vi "Initialization.vi"(8 "error in":errorcluster, 9 "UI Refs":T1, 10 "user event":T2, 11 "F18 Blowdown":refnum<class "F18 Blowdown.lvclass">) -> (0 "error out":errorcluster, 3 "F18 Blowdown OUT":refnum<class "F18 Blowdown.lvclass">)   [LabVIEW 2025, in "F18 Blowdown.lvlib" / "F18 Blowdown.lvclass"]
uses:
  F18 Blowdown.lvclass
  Users/Public/Documents/Sandia National Labs/TSS Plugin/CEF.lvlibp/Node/UserEventRef.ctl
  Users/Public/Documents/Sandia National Labs/TSS Plugin/Tests/XY Plotter.lvlibp/XY  Plotter/XY Plotter.lvclass
  F18 Blowdown.lvclass/F18 Blowdown.ctl
  Users/Public/Documents/Sandia National Labs/TSS Plugin/CEF.lvlibp/Node/CEF_Node.lvclass
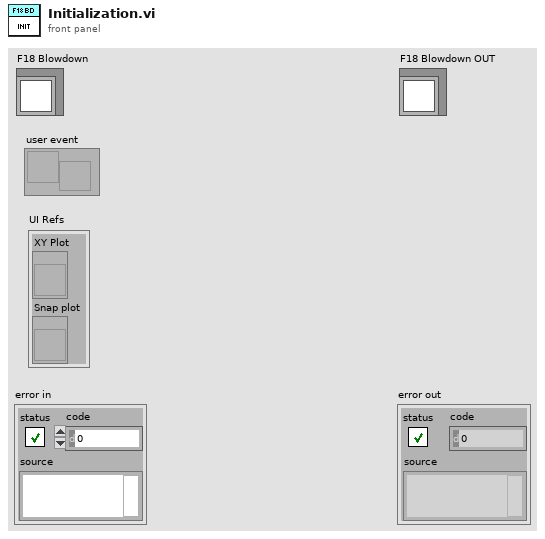
[diagram p1: front panel]
types:
  T1 = cluster{"XY Plot":refnum<vi>, "Snap plot":refnum<vi>}
  T2 = typedef "CEF.lvlibp/CEF_Node.lvclass/UserEventRef.ctl" = refnum<user-event>
  T3 = cluster{"Name":string, "Color":u32, "Style":u8, "Point Style":u8, "Name Visible":bool, "Allow Drag":bool, "Annotation Mode":u32, "Plot":i32, "Index":i32, "Position":cluster{"X":dbl, "Y":dbl}, "X Scale":u32, "Y Scale":u32, "Show Arrow":bool, "Lock Name":bool, "Plot Area":i32, "Label Offset":cluster{"X":dbl, "Y":dbl}}[]
  T4 = cluster{"Name":string, "Color":u32, "Style":u8, "Point Style":u8, "Name Visible":bool, "Allow Drag":bool, "Annotation Mode":u32, "Plot":i32, "Index":i32, "Position":cluster{"X":dbl, "Y":dbl}, "X Scale":u32, "Y Scale":u32, "Show Arrow":bool, "Lock Name":bool, "Plot Area":i32, "Label Offset":cluster{"X":dbl, "Y":dbl}}
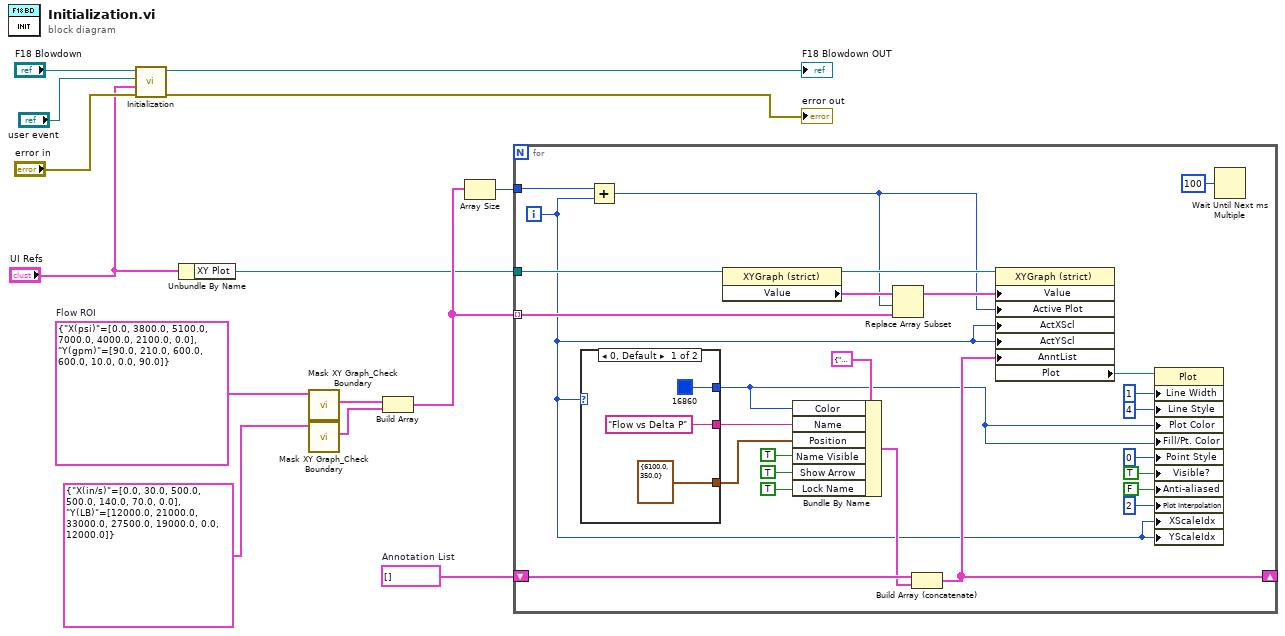
[diagram p0: block diagram]
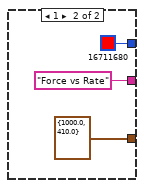
[diagram p2: hidden frame]
diagram:
  w7 = cluster{"X(psi)":dbl[], "Y(gpm)":dbl[]} {"X(psi)"=[0.0, 3800.0, 5100.0, 7000.0, 4000.0, 2100.0, 0.0], "Y(gpm)"=[90.0, 210.0, 600.0, 600.0, 10.0, 0.0, 90.0]}  # Flow ROI
  w10 = T3 []  # Annotation List
  n1 = call-parent "Initialization.vi"("error in"="error in", "UI Refs"="UI Refs", "user event"="user event", "XY Plotter"="F18 Blowdown") -> ("error out"=→"error out":errorcluster, "XY Plotter out"=→"F18 Blowdown OUT":refnum<class "F18 Blowdown.lvclass">)  [unwired: 6 in]
  n2 = Unbundle By Name("UI Refs") -> ("XY Plot"=w1:refnum<vi>)
  n3 = call "Mask XY Graph_Check Boundary.vi"("Boundary"=w7) -> ("Open Boundary"=w9:cluster{"X":dbl[], "Y":dbl[]})  [unwired: 9 in, 1 out]
  n4 = call "Mask XY Graph_Check Boundary.vi"("Boundary"=cluster{"X(in/s)":dbl[], "Y(LB)":dbl[]} {"X(in/s)"=[0.0, 30.0, 500.0, 500.0, 140.0, 70.0, 0.0], "Y(LB)"=[12000.0, 21000.0, 33000.0, 27500.0, 19000.0, 0.0, 12000.0]} ("Force ROI")) -> ("Open Boundary"=w8:cluster{"X":dbl[], "Y":dbl[]})  [unwired: 9 in, 1 out]
  n5 = Build Array(w9, w8) -> (w5:cluster{"X":dbl[], "Y":dbl[]}[])
  n6 = Array Size(array=w5) -> (size(s)=w4:i32)
  n7 = for {
    tunnel: w4 -> [w29]
    tunnel: w5 -> [w30] mode=indexing
    shift-right: [w20] -> _
    shift-left: w10 -> [w22]
    tunnel: w1 -> [w31]
    i -> [w16]
    n8 = case shown="0, Default" w16 {
      tunnel: [u32 16860 ("Plot Color") u32 16711680 ("Plot Color")] -> w19
      tunnel: ["Flow vs Delta P" ("Name") "Force vs Rate" ("Name")] -> w18
      tunnel: [cluster{"X":dbl, "Y":dbl} {"X"=6100.0, "Y"=350.0} ("Position") cluster{"X":dbl, "Y":dbl} {"X"=1000.0, "Y"=410.0} ("Position")] -> w17
      frame 0, Default {
      }
      frame 1 {
      }
    }
    n9 = Add(x=w29, y=w16) -> (x+y=w28:i32)
    n10 = property class="XYGraph (strict)"(reference=w31) -> (reference out=w38:refnum<vi>, "Value"=w39:cluster{dbl[], dbl[]}[])  [unwired: 1 in, 1 out]
    n11 = Bundle By Name(cluster=T4 {"Name"="", "Color"=0, "Style"=0, "Point Style"=0, "Name Visible"=FALSE, "Allow Drag"=FALSE, "Annotation Mode"=0, "Plot"=0, "Index"=0, "Position"={"X"=0.0, "Y"=0.0}, "X Scale"=0, "Y Scale"=0, "Show Arrow"=FALSE, "Lock Name"=FALSE, "Plot Area"=0, "Label Offset"={"X"=0.0, "Y"=0.0}}, "Color"=w19, "Name"=w18, "Position"=w17, "Name Visible"=TRUE, "Show Arrow"=TRUE, "Lock Name"=TRUE) -> (w21:T4)
    n12 = Replace Array Subset(array=w39, new element=w30, index=w28) -> (w40:cluster{dbl[], dbl[]}[])
    n13 = Build Array (concatenate)(w22, w21) -> (w20:T3)
    n14 = property class="XYGraph (strict)"(reference=w38, "Value"=w40, "Active Plot"=w28, "ActXScl"=w16, "ActYScl"=w16, "AnntList"=w20) -> ("Plot"=w27:refnum<vi>)  [unwired: 1 in, 2 out]
    n15 = property class="Plot"(reference=w27, "Line Width"=u8 1, "Line Style"=u8 4, "Plot Color"=w19, "Fill/Pt. Color"=w19, "Point Style"=u8 0, "Visible?"=TRUE ("Visible"), "Anti-aliased"=FALSE, "Plot Interpolation"=u8 2, "XScaleIdx"=w16, "YScaleIdx"=w16) -> ()  [unwired: 1 in, 2 out]
    n16 = Wait Until Next ms Multiple(millisecond multiple=u32 100) -> ()  [unwired: 1 out]
  }
